vi "usbpt104Open.vi"(1 "IP Address:port number":string="192.168.1.30:6250", 5 "Serial Number":string, 7 "Use Serial Number":bool, 8 "error in (no error)":errorcluster, 9 "Enumerate USB/Ethernet/ALL":u32(ring)=4294967295 items=["USB"=1, "Ethernet"=2, "ALL"=4294967295], 10 "Connection":bool=TRUE, 11 "SetMains":u16(ring) items=["50 Hz", "60 Hz"]) -> (0 "error out":errorcluster, 2 "Unit Info":T1, 3 "handle out":i16=16384, 4 "PT-104 Units":string, 6 "serialLth":u32=13)   [LabVIEW 2010]
doc: "This VI manages listing and opens devices with device details."
uses:
  usbpt104.dll
panel:
  # "USB"
  # "Ethernet"
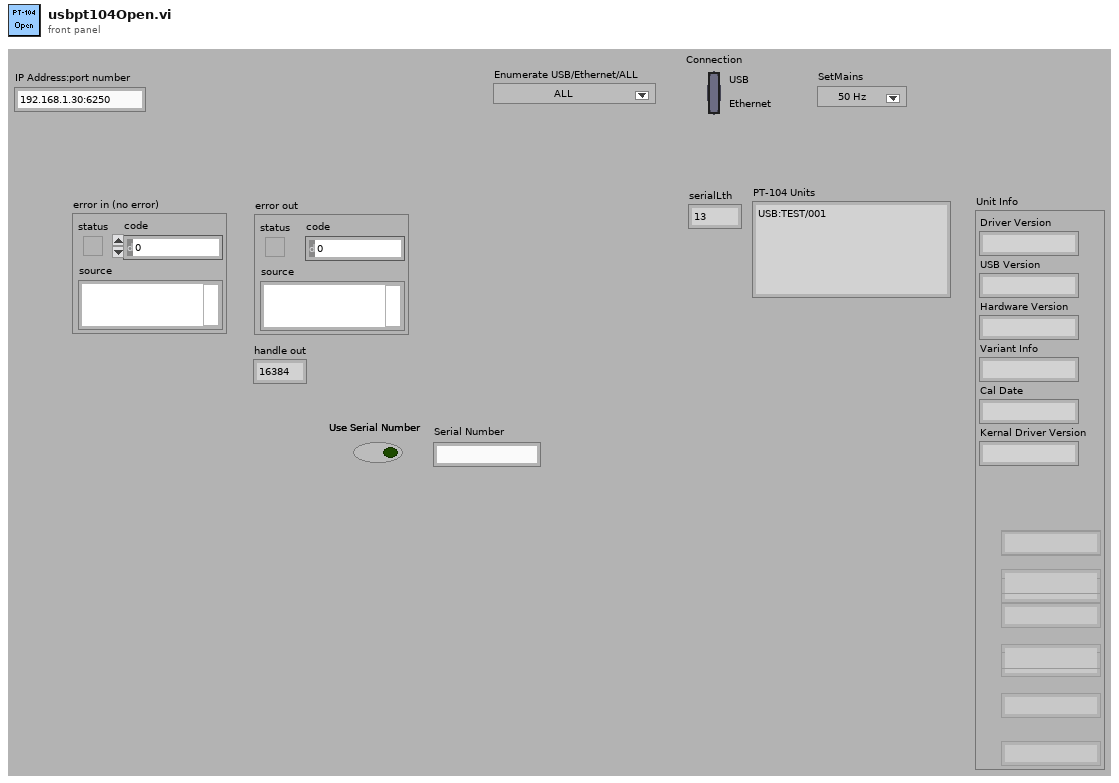
[diagram p1: front panel]
types:
  T1 = cluster{"Driver Version":string, "USB Version":string, "Hardware Version":string, "Variant Info":string, "Cal Date":string, "Kernal Driver Version":string, "NA":string, "NA 2":string, "NA":string, "NA 3":string, "NA 4":string, "NA 5":string, "NA 6":string, "NA 7":string, "NA 8":string}
  T2 = cluster{"status":bool, "code":u32, "source":string}
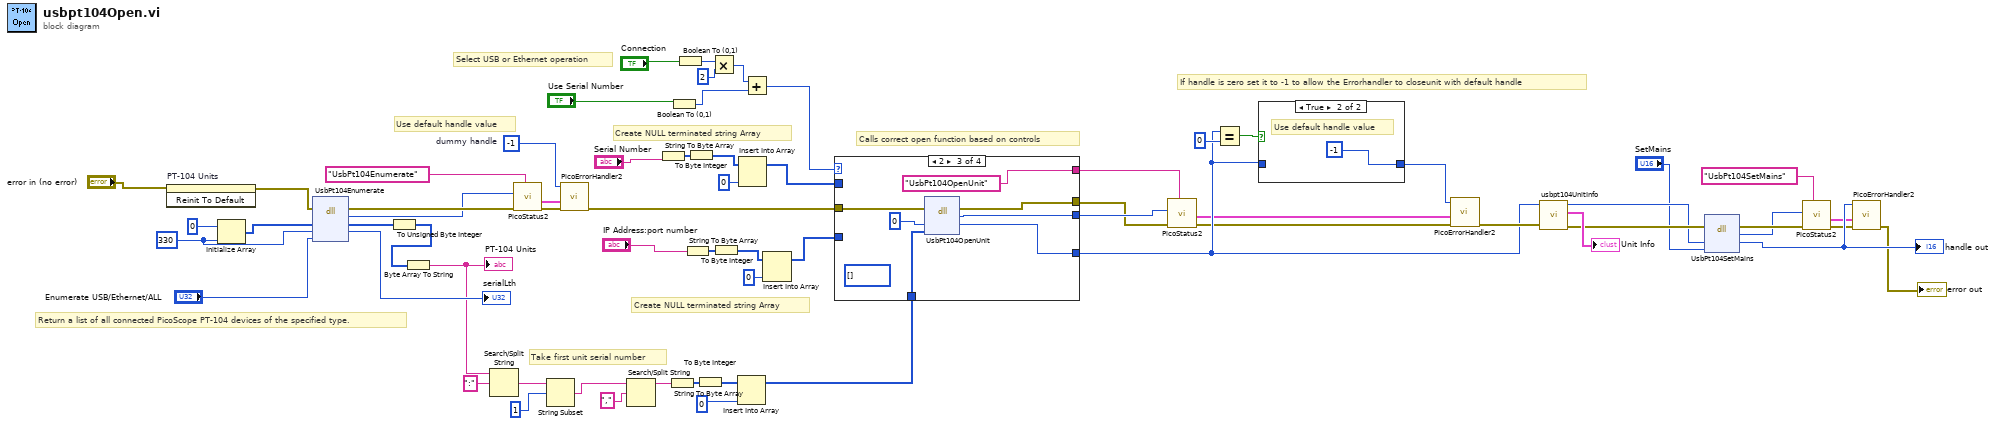
[diagram p0: block diagram]
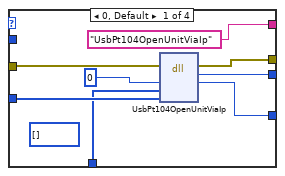
[diagram p3: hidden frame]
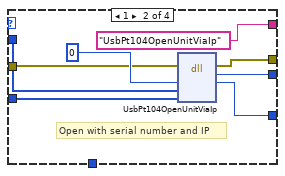
[diagram p4: hidden frame]
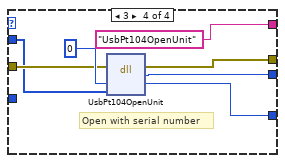
[diagram p5: hidden frame]
diagram:
  w36 = i16 -1  # dummy handle
  w53 = u32 330 ("dimension size")
  # "Take first unit serial number"
  # "If handle is zero set it to -1 to allow the Errorhandler to closeunit with default handle"
  # "Calls correct open function based on controls"
  # "Use default handle value"
  # "Create NULL terminated string Array"
  # "Create NULL terminated string Array"
  # "Return a list of all connected PicoScope PT-104 devices of the specified type."
  # "Select USB or Ethernet operation"
  n1 = invoke on="PT-104 Units" class="Str" method="Reinit To Default"(error in="error in (no error)") -> (error out=w50:errorcluster)  [unwired: 2 in, 2 out]
  n2 = Initialize Array(i8 0 ("U8"), w53) -> (w54:i8[])
  n3 = dll-call lib="UsbPT104.dll" fn="UsbPt104Enumerate"(error in=w50, "details_str"=w54, "length"=w53, "type"="Enumerate USB/Ethernet/ALL") -> (error out=w24:errorcluster, "PICO_STATUS"=w22:u32, "details_str"=w51:i8[], "length"=→"serialLth":u32)  [unwired: 3 in, 1 out]
  n4 = To Unsigned Byte Integer(number=w51) -> (unsigned 8bit integer=w52:u8[])
  n5 = Byte Array To String(unsigned byte array=w52) -> (string=w7:string)
  "PT-104 Units" <- w7
  n6 = Search/Split String(string=w7, search string/char (-)=":") -> (match + rest of string=w2:string)  [unwired: 1 in, 2 out]
  n7 = call "PicoStatus2.vi"("PICO source"="UsbPt104Enumerate" ("source"), "Error in"=w24, "PICO STATUS"=w22) -> ("error out"=w26:errorcluster, "PICO_STATUS out"=w25:T2)  [unwired: 5 in]
  n8 = String Subset(string=w2, offset (0)=1) -> (substring=w1:string)  [unwired: 1 in]
  n9 = call "PicoErrorHandler2.vi"("error in (no error)"=w26, "PICO_STATUS in"=w25, "handle In"=w36) -> ("error out"=w37:errorcluster)  [unwired: 8 in]
  n10 = Search/Split String(string=w1, search string/char (-)=",") -> (substring before match=w5:string)  [unwired: 1 in, 2 out]
  n11 = String To Byte Array(string="Serial Number") -> (unsigned byte array=w42:u8[])
  n12 = String To Byte Array(string=w5) -> (unsigned byte array=w9:u8[])
  n13 = Boolean To (0,1)(Boolean="Use Serial Number") -> (0, 1=w61:i16)
  n14 = Boolean To (0,1)(Boolean="Connection") -> (0, 1=w64:i16)
  n15 = String To Byte Array(string="IP Address:port number") -> (unsigned byte array=w47:u8[])
  n16 = To Byte Integer(number=w42) -> (8bit integer=w41:i8[])
  n17 = To Byte Integer(number=w9) -> (8bit integer=w10:i8[])
  n18 = Multiply(x=w64, y=i16 2) -> (x*y=w62:i16)
  n19 = To Byte Integer(number=w47) -> (8bit integer=w46:i8[])
  n20 = Insert Into Array(array=w10, new element=i8 0 ("new element/subarray")) -> (w4:i8[])  [unwired: 1 in]
  n21 = Insert Into Array(array=w41, new element=i8 0 ("new element/subarray")) -> (w38:i8[])  [unwired: 1 in]
  n22 = Add(x=w62, y=w61) -> (x+y=w60:i16)
  n23 = Insert Into Array(array=w46, new element=i8 0 ("new element/subarray")) -> (w43:i8[])  [unwired: 1 in]
  n24 = case shown="2" w60 {
    tunnel: [w73 w80 w88 w95] -> w18
    tunnel: [w72 w79 w86 w93] -> w32
    tunnel: [w71 w78 w87 w94] -> w17
    tunnel: w37 -> [w70 w77 w84 w91]
    tunnel: w38 -> [_ w76 _ w90]
    tunnel: w43 -> [w69 w75 _ _]
    tunnel: ["UsbPt104OpenUnitViaIp" ("source") "UsbPt104OpenUnitViaIp" ("source") "UsbPt104OpenUnit" ("source") "UsbPt104OpenUnit" ("source")] -> w19
    tunnel: w4 -> [w66 _ w82 _]
    frame 0, Default {
      (unwired) i8[] [] ("serial")
      n25 = dll-call lib="UsbPT104.dll" fn="UsbPt104OpenUnitViaIp"(error in=w70, "handle"=i16 0, "serial"=w66, "IpAddress"=w69) -> (error out=w71:errorcluster, "PICO_STATUS"=w73:u32, "handle"=w72:i16)  [unwired: 4 in, 1 out]
    }
    frame 1 {
      # "Open with serial number and IP"
      n26 = dll-call lib="UsbPT104.dll" fn="UsbPt104OpenUnitViaIp"(error in=w77, "handle"=i16 0, "serial"=w76, "IpAddress"=w75) -> (error out=w78:errorcluster, "PICO_STATUS"=w80:u32, "handle"=w79:i16)  [unwired: 4 in, 1 out]
    }
    frame 2 {
      (unwired) i8[] [] ("serial")
      n27 = dll-call lib="UsbPT104.dll" fn="UsbPt104OpenUnit"(error in=w84, "handle"=i16 0, "serial"=w82) -> (error out=w87:errorcluster, "PICO_STATUS"=w88:u32, "handle"=w86:i16)  [unwired: 3 in, 1 out]
    }
    frame 3 {
      # "Open with serial number"
      n28 = dll-call lib="UsbPT104.dll" fn="UsbPt104OpenUnit"(error in=w91, "handle"=i16 0, "serial"=w90) -> (error out=w94:errorcluster, "PICO_STATUS"=w95:u32, "handle"=w93:i16)  [unwired: 3 in, 1 out]
    }
  }
  n29 = call "PicoStatus2.vi"("PICO source"=w19, "Error in"=w17, "PICO STATUS"=w18) -> ("error out"=w21:errorcluster, "PICO_STATUS out"=w20:T2)  [unwired: 5 in]
  n30 = Equal?(x=w32, y=i16 0) -> (x = y?=w33:bool)
  n31 = case shown="True" w33 {
    tunnel: [w96 i16 -1 ("handle In")] -> w35
    tunnel: w32 -> [w96 _]
    frame False {
    }
    frame True {
      # "Use default handle value"
    }
  }
  n32 = call "PicoErrorHandler2.vi"("error in (no error)"=w21, "PICO_STATUS in"=w20, "handle In"=w35) -> ("error out"=w48:errorcluster)  [unwired: 8 in]
  n33 = call "usbpt104UnitInfo.vi"("error in (no error)"=w48, "handle in"=w32) -> ("error out"=w31:errorcluster, "Unit Info"=→"Unit Info":T1, "handle out"=w30:i16)  [unwired: 7 in]
  n34 = dll-call lib="UsbPT104.dll" fn="UsbPt104SetMains"(error in=w31, "handle"=w30, "sixty_hertz"="SetMains") -> (error out=w14:errorcluster, "PICO_STATUS"=w12:u32, "handle"=w29:i16)  [unwired: 3 in, 1 out]
  "handle out" <- w29
  n35 = call "PicoStatus2.vi"("PICO source"="UsbPt104SetMains" ("source"), "Error in"=w14, "PICO STATUS"=w12) -> ("error out"=w16:errorcluster, "PICO_STATUS out"=w15:T2)  [unwired: 5 in]
  n36 = call "PicoErrorHandler2.vi"("error in (no error)"=w16, "PICO_STATUS in"=w15, "handle In"=w29) -> ("error out"=→"error out":errorcluster)  [unwired: 8 in]
